vi "Update Data Table.vi"(10 "Output Map":T3(array[cluster]) {"OPC UA Data Type" items=["Boolean"=1, "SByte"=2, "Byte"=3, "Int16"=4, "UInt16"=5, "Int32"=6, "UInt32"=7, "Int64"=8, "UInt64"=9, "Float"=10, "Double"=11, "String"=12, "DateTime"=13, "ByteString"=15, "Array of Boolean"=101, "Array of SByte"=102, "Array of Byte"=103, "Array of Int16"=104, "Array of UInt16"=105, "Array of Int32"=106, "Array of UInt32"=107, "Array of Int64"=108, "Array of UInt64"=109, "Array of Float"=110, "Array of Double"=111, "Array of String"=112, "Array of DateTime"=113, "Array of ByteString"=115]}, 11 "data allocations":T4) -> (3 "data table out":T6)   [LabVIEW 2014, in "OPC UA Client Tests.lvlib"]
doc: "Update data table to give data allocations non-default data"
uses:
  OPC UA Client Tests.lvlib
  <vilib>/NI/Tag Bus/table/data table.ctl
  <vilib>/NI/Tag Bus Module Framework/channel/data tables.ctl
  <vilib>/NI/Tag Bus/dictionary/data dictionary.lvclass
  <vilib>/NI/Tag Bus/dictionary table pair.ctl
  <vilib>/NI/Tag Bus/tag/Data Type.ctl
  module/configuration/OPC UA Data Type.ctl
  <vilib>/NI/Tag Bus/table/data polymorphs/write one/write Double.vi
  <vilib>/NI/Tag Bus/table/data polymorphs/write one/write Single.vi
  <vilib>/NI/Tag Bus/table/data polymorphs/write one/write I64.vi
  <vilib>/NI/Tag Bus/table/data polymorphs/write one/write I32.vi
  <vilib>/NI/Tag Bus/table/data polymorphs/write one/write I16.vi
  <vilib>/NI/Tag Bus/table/data polymorphs/write one/write I8.vi
  <vilib>/NI/Tag Bus/table/data polymorphs/write one/write U64.vi
  <vilib>/NI/Tag Bus/table/data polymorphs/write one/write U32.vi
  <vilib>/NI/Tag Bus/table/data polymorphs/write one/write U16.vi
  <vilib>/NI/Tag Bus/table/data polymorphs/write one/write U8.vi
  <vilib>/NI/Tag Bus/table/data polymorphs/write one/write Boolean.vi
  <vilib>/NI/Tag Bus/table/data polymorphs/write one/write String.vi
  <vilib>/NI/Tag Bus/table/data polymorphs/write one/write Array of Double.vi
  <vilib>/NI/Tag Bus/table/data polymorphs/write one/write Array of Single.vi
  <vilib>/NI/Tag Bus/table/data polymorphs/write one/write Array of I64.vi
  <vilib>/NI/Tag Bus/table/data polymorphs/write one/write Array of I32.vi
  <vilib>/NI/Tag Bus/table/data polymorphs/write one/write Array of I16.vi
  <vilib>/NI/Tag Bus/table/data polymorphs/write one/write Array of I8.vi
  <vilib>/NI/Tag Bus/table/data polymorphs/write one/write Array of U64.vi
  <vilib>/NI/Tag Bus/table/data polymorphs/write one/write Array of U32.vi
  <vilib>/NI/Tag Bus/table/data polymorphs/write one/write Array of U16.vi
  <vilib>/NI/Tag Bus/table/data polymorphs/write one/write Array of U8.vi
  <vilib>/NI/Tag Bus/table/data polymorphs/write one/write Array of Boolean.vi
  <vilib>/NI/Tag Bus/table/data table.lvlib
  <vilib>/NI/Tag Bus/tag bus.lvlib
  <vilib>/NI/Tag Bus Module Framework/channel/TBM channel.lvclass
  <vilib>/NI/Tag Bus/tag/tag descriptor.lvclass
  module/configuration/OPC UA Client configuration.lvclass
types:
  T1 = typedef "tag bus.lvlib/tag descriptor.lvclass/Data Type.ctl" = enum16{"Double", "Single", "I64", "I32", "I16", "I8", "U64", "U32", "U16", "U8", "Boolean", "String", "Array of Double", "Array of Single", "Array of I64", "Array of I32", "Array of I16", "Array of I8", "Array of U64", "Array of U32", "Array of U16", "Array of U8", "Array of Boolean", "Array of String"}
  T2 = typedef "OPC UA Client configuration.lvclass/OPC UA Data Type.ctl" = u16
  T3 = cluster{"DCAF Data Type":T1, "Index":i32, "Node Path":string, "OPC UA Data Type":T2}[]
  T4 = typedef "TBM channel.lvclass/data tables.ctl" = cluster{"input data":T5, "processing parameter":T5, "processing result":T5, "output data":T5}
  T5 = typedef "tag bus.lvlib/dictionary table pair.ctl" = cluster{"data dictionary":refnum<class "data dictionary.lvclass">, "data table":T6}
  T6 = typedef "tag bus.lvlib/data table.lvlib/data table.ctl" = cluster{"Double":dbl[], "Single":sgl[], "I64":i64[], "I32":i32[], "I16":i16[], "I8":i8[], "U64":u64[], "U32":u32[], "U16":u16[], "U8":u8[], "Boolean":bool[], "String":string[], "Array of Double":cluster{"DBL Array":dbl[]}[], "Array of Single":cluster{"SGL Array":sgl[]}[], "Array of I64":cluster{"I64 Array":i64[]}[], "Array of I32":cluster{"I32 Array":i32[]}[], "Array of I16":cluster{"I16 Array":i16[]}[], "Array of I8":cluster{"I8 Array":i8[]}[], "Array of U64":cluster{"U64 Array":u64[]}[], "Array of U32":cluster{"U32 Array":u32[]}[], "Array of U16":cluster{"U16 Array":u16[]}[], "Array of U8":cluster{"U8 Array":u8[]}[], "Array of Boolean":cluster{"Boolean Array":bool[]}[], "Array of String":cluster{"String Array":string[]}[]}
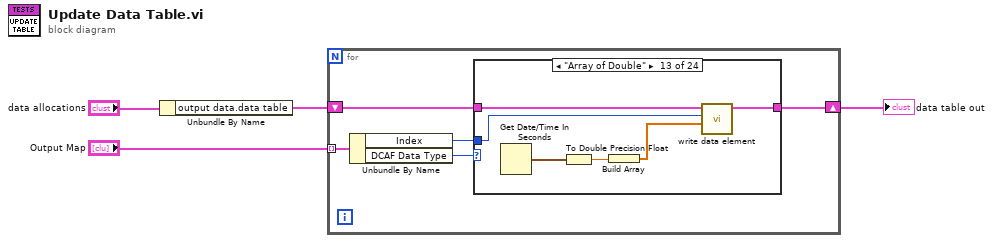
[diagram p0: block diagram]
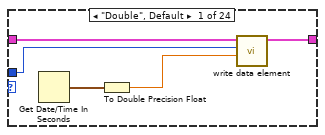
[diagram p2: hidden frame]
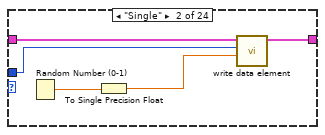
[diagram p3: hidden frame]
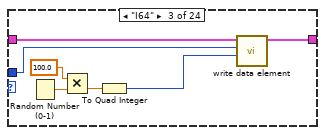
[diagram p4: hidden frame]
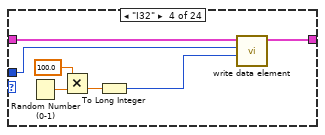
[diagram p5: hidden frame]
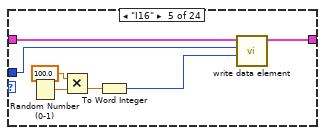
[diagram p6: hidden frame]
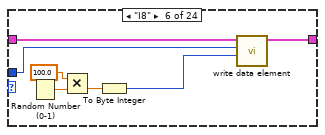
[diagram p7: hidden frame]
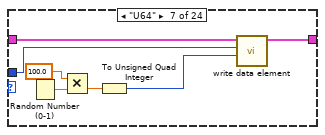
[diagram p8: hidden frame]
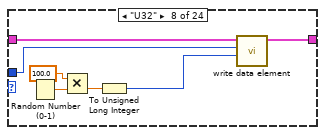
[diagram p9: hidden frame]
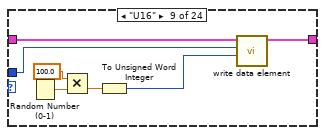
[diagram p10: hidden frame]
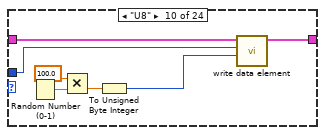
[diagram p11: hidden frame]
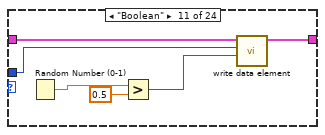
[diagram p12: hidden frame]
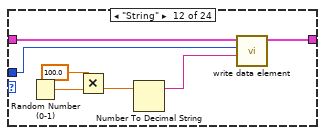
[diagram p13: hidden frame]
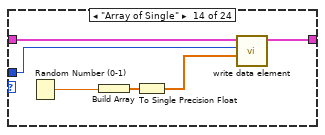
[diagram p14: hidden frame]
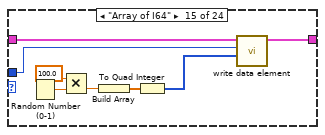
[diagram p15: hidden frame]
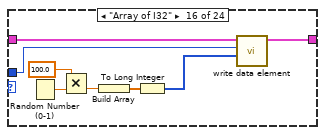
[diagram p16: hidden frame]
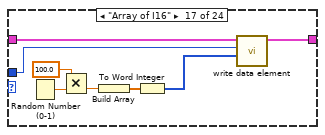
[diagram p17: hidden frame]
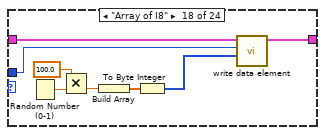
[diagram p18: hidden frame]
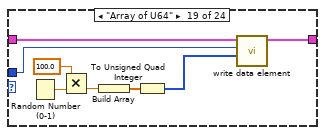
[diagram p19: hidden frame]
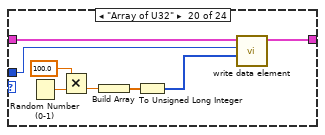
[diagram p20: hidden frame]
diagram:
  n1 = Unbundle By Name("data allocations") -> ("output data.data table"=w2:T6)
  n2 = for {
    tunnel: "Output Map" -> [w9] mode=indexing
    shift-right: [w7] -> w1
    shift-left: w2 -> [w6]
    n3 = Unbundle By Name(w9) -> ("Index"=w5:i32, "DCAF Data Type"=w8:T1)
    n4 = case shown="\"Array of Double\"" w8 {
      tunnel: [w14 w19 w26 w33 w40 w47 w54 w61 w68 w75 w81 w88 w94 w100 w108 w116 w124 w132 w140 w148 w156 w164 w171 w178] -> w7
      tunnel: w6 -> [w13 w18 w25 w32 w39 w46 w53 w60 w67 w74 w80 w87 w93 w99 w107 w115 w123 w131 w139 w147 w155 w163 w170 w177]
      tunnel: w5 -> [w12 w16 w23 w30 w37 w44 w51 w58 w65 w72 w79 w85 w92 w97 w105 w113 w121 w129 w137 w145 w153 w161 w169 w176]
      frame "Double", Default {
        n5 = Get Date/Time In Seconds() -> (seconds since 1Jan1904=w11:timestamp)
        n6 = To Double Precision Float(number=w11) -> (double precision float=w10:dbl)
        n7 = call-poly <vilib>:"write data element.vi"("value"=w10, "index"=w12, "data table in"=w13) -> ("data table out"=w14:T6)  [unwired: 8 in]
      }
      frame "Single" {
        n8 = Random Number (0-1)() -> (number: 0 to 1=w17:dbl)
        n9 = To Single Precision Float(number=w17) -> (single precision float=w15:sgl)
        n10 = call-poly <vilib>:"write data element.vi"("value"=w15, "index"=w16, "data table in"=w18) -> ("data table out"=w19:T6)  [unwired: 8 in]
      }
      frame "I64" {
        n11 = Random Number (0-1)() -> (number: 0 to 1=w24:dbl)
        n12 = Multiply(x=100.0, y=w24) -> (x*y=w21:dbl)
        n13 = To Quad Integer(1:w21) -> (0:w22:i64)
        n14 = call-poly <vilib>:"write data element.vi"("value"=w22, "index"=w23, "data table in"=w25) -> ("data table out"=w26:T6)  [unwired: 8 in]
      }
      frame "I32" {
        n15 = Random Number (0-1)() -> (number: 0 to 1=w31:dbl)
        n16 = Multiply(x=100.0, y=w31) -> (x*y=w28:dbl)
        n17 = To Long Integer(number=w28) -> (32bit integer=w29:i32)
        n18 = call-poly <vilib>:"write data element.vi"("value"=w29, "index"=w30, "data table in"=w32) -> ("data table out"=w33:T6)  [unwired: 8 in]
      }
      frame "I16" {
        n19 = Random Number (0-1)() -> (number: 0 to 1=w38:dbl)
        n20 = Multiply(x=100.0, y=w38) -> (x*y=w35:dbl)
        n21 = To Word Integer(number=w35) -> (16bit integer=w36:i16)
        n22 = call-poly <vilib>:"write data element.vi"("value"=w36, "index"=w37, "data table in"=w39) -> ("data table out"=w40:T6)  [unwired: 8 in]
      }
      frame "I8" {
        n23 = Random Number (0-1)() -> (number: 0 to 1=w45:dbl)
        n24 = Multiply(x=100.0, y=w45) -> (x*y=w42:dbl)
        n25 = To Byte Integer(number=w42) -> (8bit integer=w43:i8)
        n26 = call-poly <vilib>:"write data element.vi"("value"=w43, "index"=w44, "data table in"=w46) -> ("data table out"=w47:T6)  [unwired: 8 in]
      }
      frame "U64" {
        n27 = Random Number (0-1)() -> (number: 0 to 1=w52:dbl)
        n28 = Multiply(x=100.0, y=w52) -> (x*y=w49:dbl)
        n29 = To Unsigned Quad Integer(1:w49) -> (0:w50:u64)
        n30 = call-poly <vilib>:"write data element.vi"("value"=w50, "index"=w51, "data table in"=w53) -> ("data table out"=w54:T6)  [unwired: 8 in]
      }
      frame "U32" {
        n31 = Random Number (0-1)() -> (number: 0 to 1=w59:dbl)
        n32 = Multiply(x=100.0, y=w59) -> (x*y=w56:dbl)
        n33 = To Unsigned Long Integer(number=w56) -> (unsigned 32bit integer=w57:u32)
        n34 = call-poly <vilib>:"write data element.vi"("value"=w57, "index"=w58, "data table in"=w60) -> ("data table out"=w61:T6)  [unwired: 8 in]
      }
      frame "U16" {
        n35 = Random Number (0-1)() -> (number: 0 to 1=w66:dbl)
        n36 = Multiply(x=100.0, y=w66) -> (x*y=w63:dbl)
        n37 = To Unsigned Word Integer(number=w63) -> (unsigned 16bit integer=w64:u16)
        n38 = call-poly <vilib>:"write data element.vi"("value"=w64, "index"=w65, "data table in"=w67) -> ("data table out"=w68:T6)  [unwired: 8 in]
      }
      frame "U8" {
        n39 = Random Number (0-1)() -> (number: 0 to 1=w73:dbl)
        n40 = Multiply(x=100.0, y=w73) -> (x*y=w70:dbl)
        n41 = To Unsigned Byte Integer(number=w70) -> (unsigned 8bit integer=w71:u8)
        n42 = call-poly <vilib>:"write data element.vi"("value"=w71, "index"=w72, "data table in"=w74) -> ("data table out"=w75:T6)  [unwired: 8 in]
      }
      frame "Boolean" {
        n43 = Random Number (0-1)() -> (number: 0 to 1=w77:dbl)
        n44 = Greater?(x=w77, y=0.5) -> (0:w78:bool)
        n45 = call-poly <vilib>:"write data element.vi"("value"=w78, "index"=w79, "data table in"=w80) -> ("data table out"=w81:T6)  [unwired: 8 in]
      }
      frame "String" {
        n46 = Random Number (0-1)() -> (number: 0 to 1=w86:dbl)
        n47 = Multiply(x=100.0, y=w86) -> (x*y=w83:dbl)
        n48 = Number To Decimal String(number=w83) -> (decimal integer string=w84:string)  [unwired: 1 in]
        n49 = call-poly <vilib>:"write data element.vi"("value"=w84, "index"=w85, "data table in"=w87) -> ("data table out"=w88:T6)  [unwired: 8 in]
      }
      frame "Array of Double" {
        n50 = Get Date/Time In Seconds() -> (seconds since 1Jan1904=w91:timestamp)
        n51 = To Double Precision Float(number=w91) -> (double precision float=w90:dbl)
        n52 = Build Array(w90) -> (w89:dbl[])
        n53 = call-poly <vilib>:"write data element.vi"("value"=w89, "index"=w92, "data table in"=w93) -> ("data table out"=w94:T6)  [unwired: 8 in]
      }
      frame "Array of Single" {
        n54 = Random Number (0-1)() -> (number: 0 to 1=w98:dbl)
        n55 = Build Array(w98) -> (w96:dbl[])
        n56 = To Single Precision Float(number=w96) -> (single precision float=w95:sgl[])
        n57 = call-poly <vilib>:"write data element.vi"("value"=w95, "index"=w97, "data table in"=w99) -> ("data table out"=w100:T6)  [unwired: 8 in]
      }
      frame "Array of I64" {
        n58 = Random Number (0-1)() -> (number: 0 to 1=w106:dbl)
        n59 = Multiply(x=100.0, y=w106) -> (x*y=w102:dbl)
        n60 = Build Array(w102) -> (w104:dbl[])
        n61 = To Quad Integer(1:w104) -> (0:w103:i64[])
        n62 = call-poly <vilib>:"write data element.vi"("value"=w103, "index"=w105, "data table in"=w107) -> ("data table out"=w108:T6)  [unwired: 8 in]
      }
      frame "Array of I32" {
        n63 = Random Number (0-1)() -> (number: 0 to 1=w114:dbl)
        n64 = Multiply(x=100.0, y=w114) -> (x*y=w110:dbl)
        n65 = Build Array(w110) -> (w112:dbl[])
        n66 = To Long Integer(number=w112) -> (32bit integer=w111:i32[])
        n67 = call-poly <vilib>:"write data element.vi"("value"=w111, "index"=w113, "data table in"=w115) -> ("data table out"=w116:T6)  [unwired: 8 in]
      }
      frame "Array of I16" {
        n68 = Random Number (0-1)() -> (number: 0 to 1=w122:dbl)
        n69 = Multiply(x=100.0, y=w122) -> (x*y=w118:dbl)
        n70 = Build Array(w118) -> (w120:dbl[])
        n71 = To Word Integer(number=w120) -> (16bit integer=w119:i16[])
        n72 = call-poly <vilib>:"write data element.vi"("value"=w119, "index"=w121, "data table in"=w123) -> ("data table out"=w124:T6)  [unwired: 8 in]
      }
      frame "Array of I8" {
        n73 = Random Number (0-1)() -> (number: 0 to 1=w130:dbl)
        n74 = Multiply(x=100.0, y=w130) -> (x*y=w126:dbl)
        n75 = Build Array(w126) -> (w128:dbl[])
        n76 = To Byte Integer(number=w128) -> (8bit integer=w127:i8[])
        n77 = call-poly <vilib>:"write data element.vi"("value"=w127, "index"=w129, "data table in"=w131) -> ("data table out"=w132:T6)  [unwired: 8 in]
      }
      frame "Array of U64" {
        n78 = Random Number (0-1)() -> (number: 0 to 1=w138:dbl)
        n79 = Multiply(x=100.0, y=w138) -> (x*y=w134:dbl)
        n80 = Build Array(w134) -> (w136:dbl[])
        n81 = To Unsigned Quad Integer(1:w136) -> (0:w135:u64[])
        n82 = call-poly <vilib>:"write data element.vi"("value"=w135, "index"=w137, "data table in"=w139) -> ("data table out"=w140:T6)  [unwired: 8 in]
      }
      frame "Array of U32" {
        n83 = Random Number (0-1)() -> (number: 0 to 1=w146:dbl)
        n84 = Multiply(x=100.0, y=w146) -> (x*y=w142:dbl)
        n85 = Build Array(w142) -> (w144:dbl[])
        n86 = To Unsigned Long Integer(number=w144) -> (unsigned 32bit integer=w143:u32[])
        n87 = call-poly <vilib>:"write data element.vi"("value"=w143, "index"=w145, "data table in"=w147) -> ("data table out"=w148:T6)  [unwired: 8 in]
      }
      frame "Array of U16" {
        n88 = Random Number (0-1)() -> (number: 0 to 1=w154:dbl)
        n89 = Multiply(x=100.0, y=w154) -> (x*y=w150:dbl)
        n90 = Build Array(w150) -> (w152:dbl[])
        n91 = To Unsigned Word Integer(number=w152) -> (unsigned 16bit integer=w151:u16[])
        n92 = call-poly <vilib>:"write data element.vi"("value"=w151, "index"=w153, "data table in"=w155) -> ("data table out"=w156:T6)  [unwired: 8 in]
      }
      frame "Array of U8" {
        n93 = Random Number (0-1)() -> (number: 0 to 1=w162:dbl)
        n94 = Multiply(x=100.0, y=w162) -> (x*y=w158:dbl)
        n95 = Build Array(w158) -> (w160:dbl[])
        n96 = To Unsigned Byte Integer(number=w160) -> (unsigned 8bit integer=w159:u8[])
        n97 = call-poly <vilib>:"write data element.vi"("value"=w159, "index"=w161, "data table in"=w163) -> ("data table out"=w164:T6)  [unwired: 8 in]
      }
      frame "Array of Boolean" {
        n98 = Random Number (0-1)() -> (number: 0 to 1=w168:dbl)
        n99 = Greater?(x=w168, y=0.5) -> (0:w166:bool)
        n100 = Build Array(w166) -> (w165:bool[])
        n101 = call-poly <vilib>:"write data element.vi"("value"=w165, "index"=w169, "data table in"=w170) -> ("data table out"=w171:T6)  [unwired: 8 in]
      }
      frame "Array of String" {
        n102 = Random Number (0-1)() -> (number: 0 to 1=w175:dbl)
        n103 = Multiply(x=100.0, y=w175) -> (x*y=w173:dbl)
        n104 = Build Array(w173) -> (w172:dbl[])
        n105 = call-poly <vilib>:"write data element.vi"("value"=w172, "index"=w176, "data table in"=w177) -> ("data table out"=w178:T6)  [unwired: 8 in]
      }
    }
  }
  "data table out" <- w1
